vi "RemoteVI Publish Status.vi"(0 "info":T3, 1 "started":dbl, 2 "clients":T2(array[cluster]), 3 "captured?":bool, 5 "clicked?":bool, 7 "error":errorcluster, 8 "stop?":bool, 9 "state":T1, 10 "hWnd":u64) -> (4 "state out":T1)   [LabVIEW 2020, in "RemoteVI.lvlib"]
doc: "Keeps the server loop's statistics and publishes its status (RemoteVI Status Registry.vi) every 500 ms: frames counts the frames made (captured?); fps and bytes per s are the frames made and the bytes sent to all clients (the clients' bytes) per second since the last publication; latency ms is the time from the iteration of the last remote click or key (clicked?) to the next frame made after it. The entry carries info (port, link with token, target, kind, whole network, view only), started, the time of this publication (updated), every client's address, connected since and last input, and the source of error when it carries one. With stop? TRUE the entry is removed instead (the server loop ends). Times are seconds since the LabVIEW epoch. No VI Server call."
uses:
  RemoteVI.lvlib
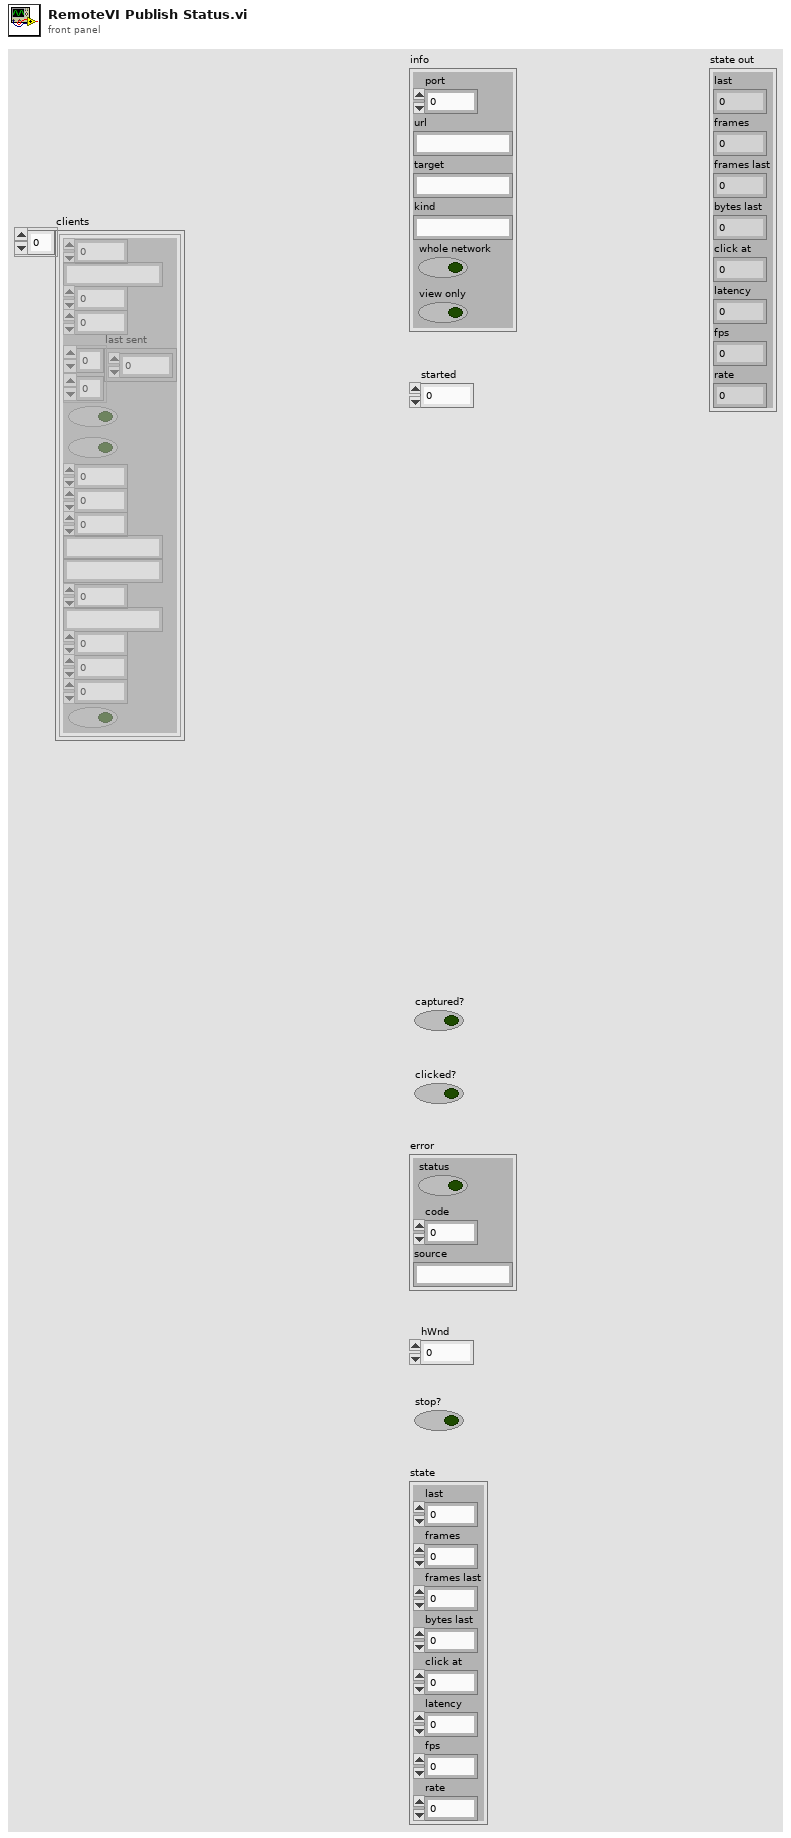
[diagram p1: front panel]
types:
  T1 = cluster{"last":dbl, "frames":u32, "frames last":u32, "bytes last":dbl, "click at":dbl, "latency":dbl, "fps":dbl, "rate":dbl}
  T2 = cluster{"connection":u32, "rx buffer":string, "seq":u32, "acked":u32, "last sent":u32[][], "tracking":bool, "closed":bool, "mods":u8, "mods set":u8, "popup since":u32, "windows sent":string, "window frames":cluster{"id":u64, "pixels":u32[][]}[], "key window":u64, "address":string, "since":dbl, "last input":dbl, "bytes":dbl, "view only":bool}[]
  T3 = cluster{"port":u16, "url":string, "target":string, "kind":string, "whole network":bool, "view only":bool}
  T4 = cluster{"address":string, "since":dbl, "last input":dbl}
  T5 = cluster{"port":u16, "url":string, "target":string, "kind":string, "whole network":bool, "started":dbl, "updated":dbl, "clients":cluster{"address":string, "since":dbl, "last input":dbl}[], "fps":dbl, "bytes per s":dbl, "frames":u32, "latency ms":dbl, "view only":bool, "last error":string, "hWnd":u64}
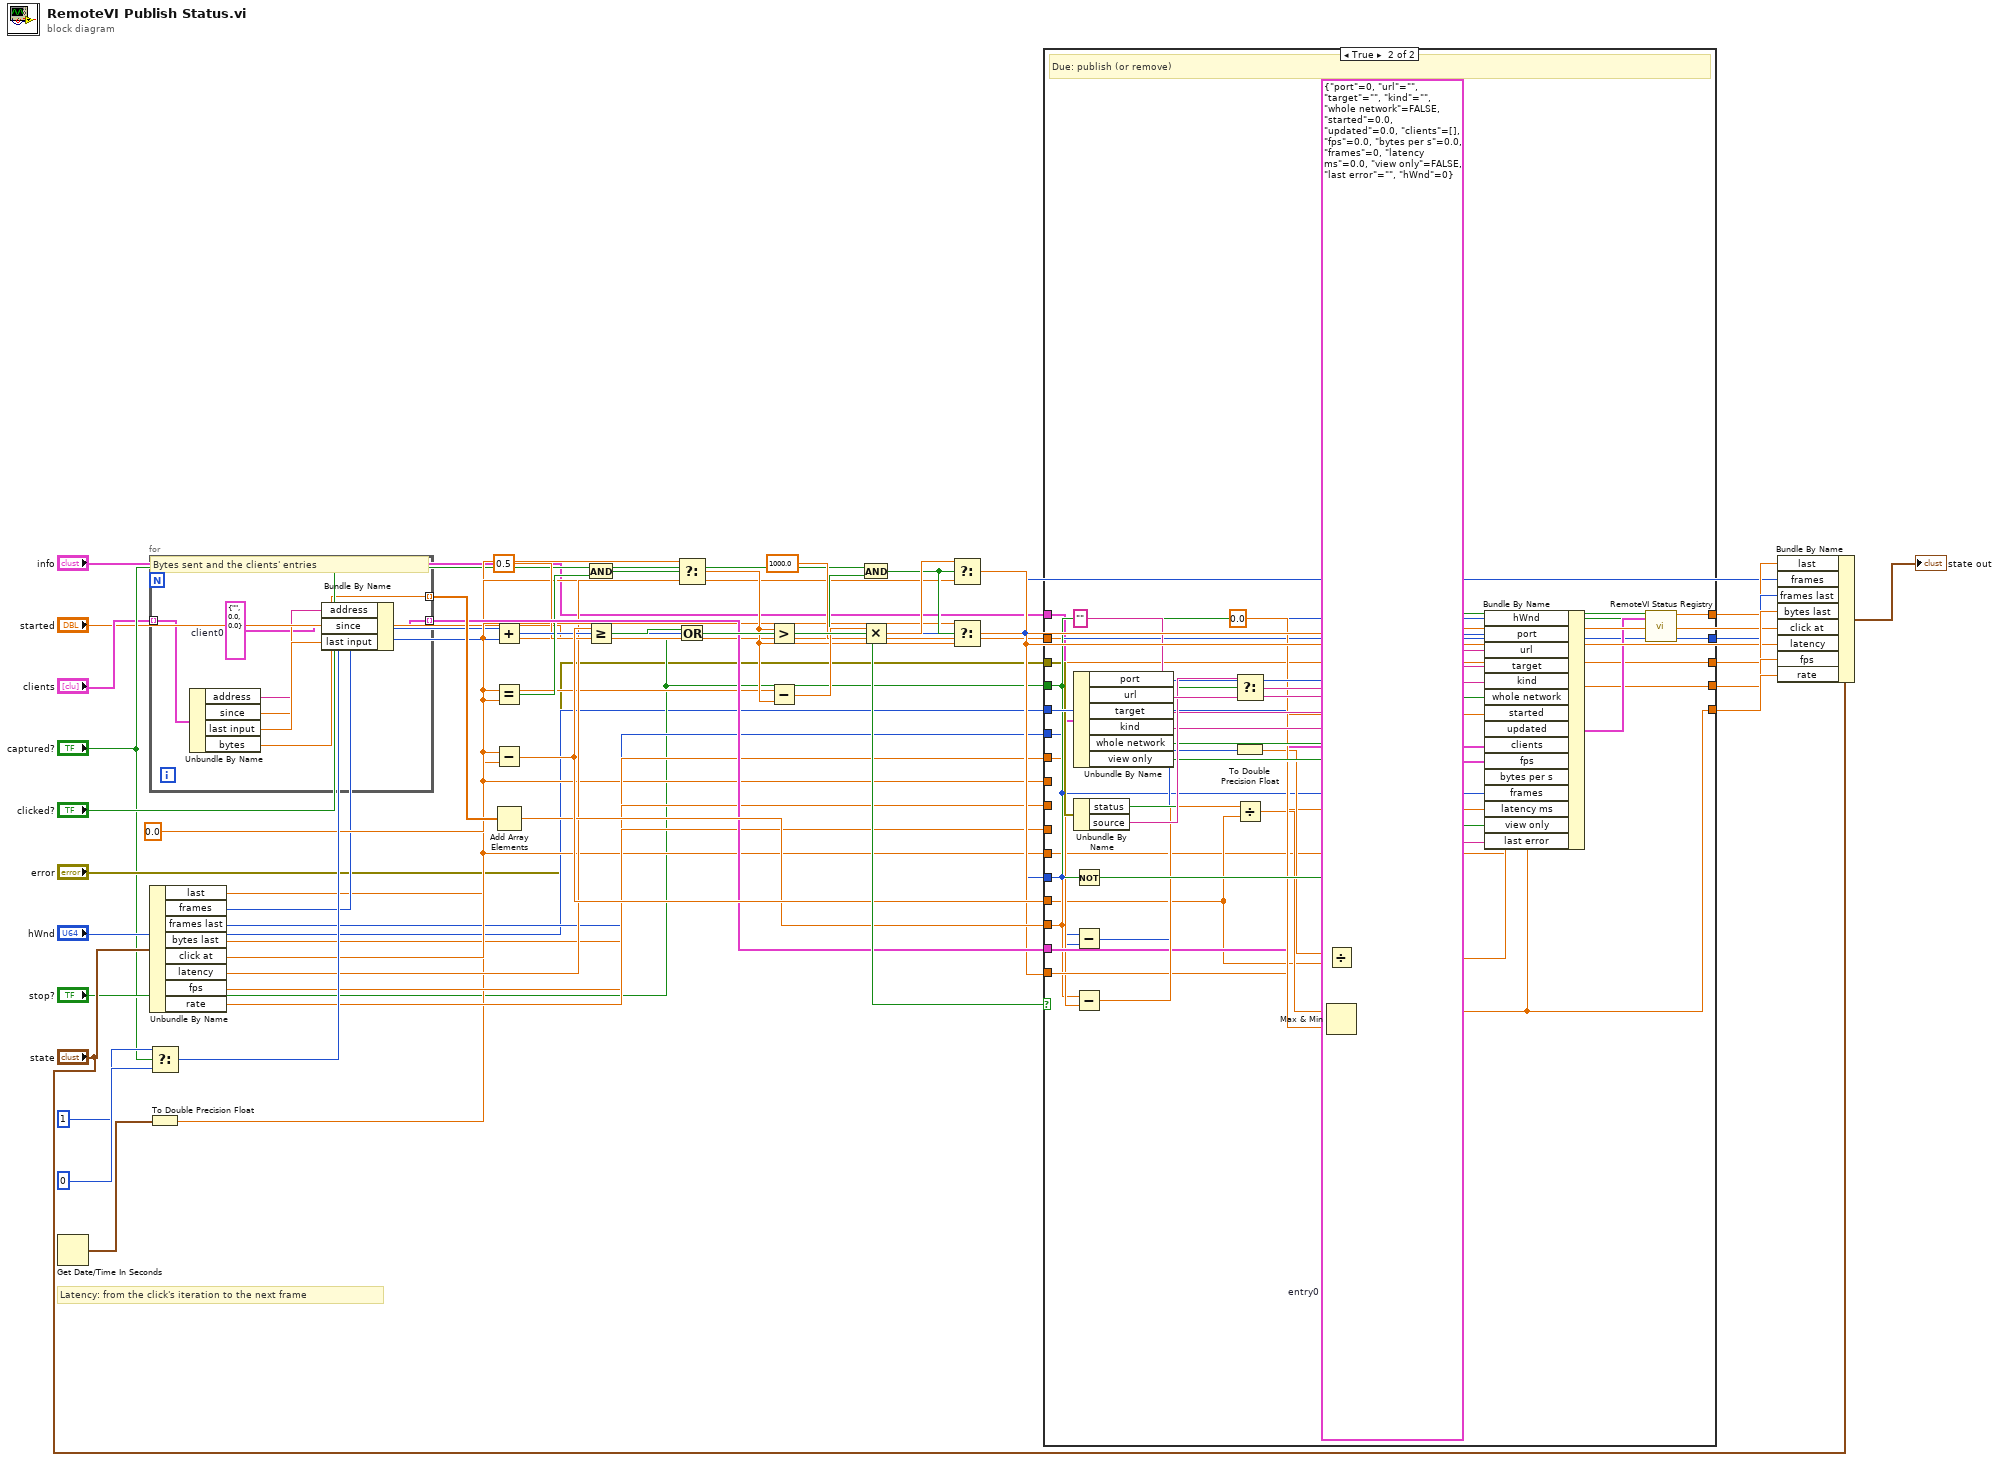
[diagram p0: block diagram]
diagram:
  w22 = 0.0
  # "Latency: from the click's iteration to the next frame"
  n1 = Get Date/Time In Seconds() -> (seconds since 1Jan1904=w10:timestamp)
  n2 = for {
    tunnel: "clients" -> [w48] mode=indexing
    tunnel: [w53] -> w37 mode=indexing
    tunnel: [w54] -> w36 mode=indexing
    w49 = T4 {"address"="", "since"=0.0, "last input"=0.0}  # client0
    # "Bytes sent and the clients' entries"
    n3 = Unbundle By Name(w48) -> ("address"=w50:string, "since"=w51:dbl, "last input"=w52:dbl, "bytes"=w53:dbl)
    n4 = Bundle By Name(cluster=w49, "address"=w50, "since"=w51, "last input"=w52) -> (w54:T4)
  }
  n5 = Unbundle By Name("state") -> ("last"=w12:dbl, "frames"=w13:u32, "frames last"=w14:u32, "bytes last"=w15:dbl, "click at"=w16:dbl, "latency"=w17:dbl, "fps"=w18:dbl, "rate"=w19:dbl)
  n6 = Select(t=u32 1, s="captured?", f=u32 0) -> (s? t:f=w25:u32)
  n7 = To Double Precision Float(number=w10) -> (double precision float=w11:dbl)
  n8 = Add(x=w13, y=w25) -> (x+y=w26:u32)
  n9 = Equal?(x=w16, y=w22) -> (x = y?=w27:bool)
  n10 = Subtract(x=w11, y=w12) -> (x-y=w39:dbl)
  n11 = Add Array Elements(numeric array=w37) -> (sum=w38:dbl)
  n12 = And(x="clicked?", y=w27) -> (x .and. y?=w28:bool)
  n13 = Greater Or Equal?(x=w39, y=0.5) -> (x >= y?=w40:bool)
  n14 = Select(t=w11, s=w28, f=w16) -> (s? t:f=w29:dbl)
  n15 = Or(x=w40, y="stop?") -> (x .or. y?=w41:bool)
  n16 = Greater?(x=w29, y=w22) -> (0:w30:bool)
  n17 = Subtract(x=w11, y=w29) -> (x-y=w32:dbl)
  n18 = And(x="captured?", y=w30) -> (x .and. y?=w31:bool)
  n19 = Multiply(x=w32, y=1000.0) -> (x*y=w33:dbl)
  n20 = Select(t=w33, s=w31, f=w17) -> (s? t:f=w34:dbl)
  n21 = Select(t=w22, s=w31, f=w29) -> (s? t:f=w35:dbl)
  n22 = case shown="True" w41 {
    tunnel: "info" -> [_ w60]
    tunnel: "started" -> [_ w61]
    tunnel: "error" -> [_ w70]
    tunnel: "stop?" -> [_ w71]
    tunnel: "hWnd" -> [_ w72]
    tunnel: w14 -> [w55 w65]
    tunnel: w15 -> [w56 w67]
    tunnel: w12 -> [w57 _]
    tunnel: w18 -> [w58 _]
    tunnel: w19 -> [w59 _]
    tunnel: w11 -> [_ w62]
    tunnel: w26 -> [_ w64]
    tunnel: w39 -> [_ w63]
    tunnel: [w57 w62] -> w42
    tunnel: [w55 w64] -> w43
    tunnel: w38 -> [_ w66]
    tunnel: w36 -> [_ w68]
    tunnel: [w56 w66] -> w44
    tunnel: [w58 w75] -> w45
    tunnel: w34 -> [_ w69]
    tunnel: [w59 w79] -> w46
    frame False {
      # "Not yet"
    }
    frame True {
      w90 = T5 {"port"=0, "url"="", "target"="", "kind"="", "whole network"=FALSE, "started"=0.0, "updated"=0.0, "clients"=[], "fps"=0.0, "bytes per s"=0.0, "frames"=0, "latency ms"=0.0, "view only"=FALSE, "last error"="", "hWnd"=0}  # entry0
      # "Due: publish (or remove)"
      n23 = Unbundle By Name(w60) -> ("port"=w80:u16, "url"=w81:string, "target"=w82:string, "kind"=w83:string, "whole network"=w84:bool, "view only"=w85:bool)
      n24 = Unbundle By Name(w70) -> ("status"=w86:bool, "source"=w87:string)
      n25 = Not(x=w71) -> (.not. x?=w92:bool)
      n26 = Subtract(x=w64, y=w65) -> (x-y=w73:u32)
      n27 = Subtract(x=w66, y=w67) -> (x-y=w76:dbl)
      n28 = Select(t=w87, s=w86, f="") -> (s? t:f=w89:string)
      n29 = To Double Precision Float(number=w73) -> (double precision float=w74:dbl)
      n30 = Divide(x=w76, y=w63) -> (x/y=w77:dbl)
      n31 = Divide(x=w74, y=w63) -> (x/y=w75:dbl)
      n32 = Max & Min(x=w77, y=0.0) -> (max(x,y)=w79:dbl)  [unwired: 1 out]
      n33 = Bundle By Name(cluster=w90, "hWnd"=w72, "port"=w80, "url"=w81, "target"=w82, "kind"=w83, "whole network"=w84, "started"=w61, "updated"=w62, "clients"=w68, "fps"=w75, "bytes per s"=w79, "frames"=w64, "latency ms"=w69, "view only"=w85, "last error"=w89) -> (w91:T5)
      n34 = call "RemoteVI Status Registry.vi"("publish?"=w92, "remove?"=w71, "status"=w91) -> ()  [unwired: 12 in, 1 out]
    }
  }
  n35 = Bundle By Name(cluster="state", "last"=w42, "frames"=w26, "frames last"=w43, "bytes last"=w44, "click at"=w35, "latency"=w34, "fps"=w45, "rate"=w46) -> (→"state out":T1)
